vi "getLinkFrequency.vi"(8 "error in (no error)":errorcluster, 11 "Instrument.Lockin in":refnum<class "Instrument.Lockin.lvclass">) -> (0 "error out":errorcluster, 1 "Frequency (Hz)":dbl=13.0, 2 "Link?":bool, 3 "Instrument.Lockin out":refnum<class "Instrument.Lockin.lvclass">)   [LabVIEW 2019, in "Instrument.Lockin.lvlib" / "Instrument.Lockin.lvclass"]
doc: "API to configure a REF frequency.\n\nSpecify which channel you want to change and the value you want to set.\n\nIf address=\"\", this API reads from localhost\nIf address is remote lockin, you need to add this computer to allowed whitelist on the lockin computer you are trying to access."
uses:
  Instrument.Lockin.lvclass
  Lockin.Typedefs/API/Lockin.Commands--Enum.ctl
  Lockin.Typedefs/Configuration/Configuration.LinkFrequencies--Cluster.ctl
  59998681-cfc0-40a9-8474-49d1772e29ea.vi
  <vilib>/PRIrvin/JSON-RPC/API/JSON to Variant.vi
  <vilib>/Utility/Data Type/Get Type Information.vi
  <vilib>/JDP Science/JSONtext/JSON type.vi
  <vilib>/JDP Science/JSONtext/Get Array Elements.vi
  <vilib>/JDP Science/JSONtext/JSON text to Variant.vi
  Lockin.Typedefs/Lockin.Typedefs.lvlib
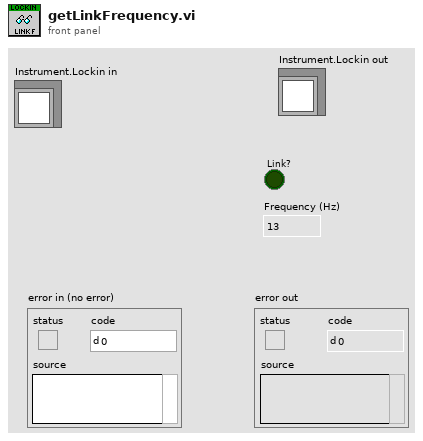
[diagram p1: front panel]
types:
  T1 = typedef "Lockin.Typedefs.lvlib/Configuration.LinkFrequencies--Cluster.ctl" = cluster{"Link":bool, "Frequency":dbl}
  T2 = typedef "Lockin.Typedefs.lvlib/Lockin.Commands--Enum.ctl" = enum16{"setAO", "setAO_Amplitude", "setAO_DC", "setAO_Frequency", "setAO_Phase", "setAO_Function", "setREF", "setREF_Frequency", "setREF_Phase", "setREF_TC", "setREF_Roll-Off", "setDAQ", "setSampling", "setState", "getState", "getAO", "getAI", "getResults", "getSampling", "getAOconfig", "getREFconfig", "setInputGain", "setOutputGain", "getInputGain", "getOutputGain", "setSweep", "setSweepTime", "setSweepTable", "getStatus", "getSweepResults", "getSweepWaveforms", "logConfiguration", "startLogging", "stopLogging", "setInputOffset", "getInputOffset", "setOutputOffset", "getOutputOffset", "getInputDAQ", "getOutputDAQ", "getLinkFrequency", "setLinkFrequency", "measureInputOffset", "getDevices"}
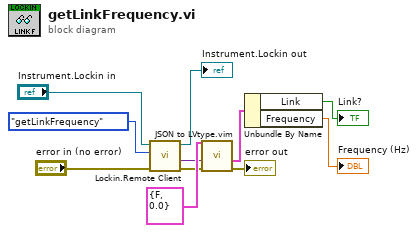
[diagram p0: block diagram]
diagram:
  n1 = call "Lockin.Remote Client.vi"("error in (no error)"="error in (no error)", "Command"=Lockin.Commands--Enum."getLinkFrequency" ("Enum"), "Instrument.Lockin in"="Instrument.Lockin in") -> ("error out"=w3:errorcluster, "Data out"=w4:variant, "Instrument.Lockin out"=→"Instrument.Lockin out":refnum<class "Instrument.Lockin.lvclass">)  [unwired: 6 in]
  n2 = call "JSON to LVtype.vim"("type"=T1 {"Link"=FALSE, "Frequency"=0.0} ("Link Frequencies"), "error in (no error)"=w3, "JSON Data in"=w4) -> ("error out"=→"error out":errorcluster, "Data out"=w1:T1)  [unwired: 7 in]
  n3 = Unbundle By Name(w1) -> ("Link"=→"Link?":bool, "Frequency"=→"Frequency (Hz)":dbl)
